vi "lvmcp_termctl.vi"() -> ()   [LabVIEW 2026]
panel:
  out "error out":errorcluster
  in  "reference":refnum<vi>
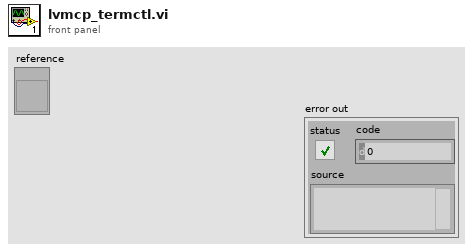
[diagram p1: front panel]
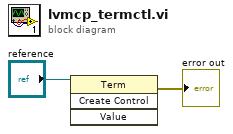
[diagram p0: block diagram]
diagram:
  n1 = invoke class="Term" method="Create Control"(reference="reference") -> (error out=→"error out":errorcluster)  [unwired: 3 in, 3 out]
